vi "Get Summary.vi"(7 "Style":enum16{"Diff", "Plain"}(ring), 8 "error in (no error)":errorcluster, 10 "Item":string, 11 "Result Model by Reference In":refnum<class "Result Model.lvclass">) -> (0 "error out":errorcluster, 2 "Summary":string)   [LabVIEW 2020, in "Result Model.lvclass"]
uses:
  Result Model.lvclass
  Result Model.lvclass/Result Model.ctl
  Framework/Utilities/Utilities.lvlib
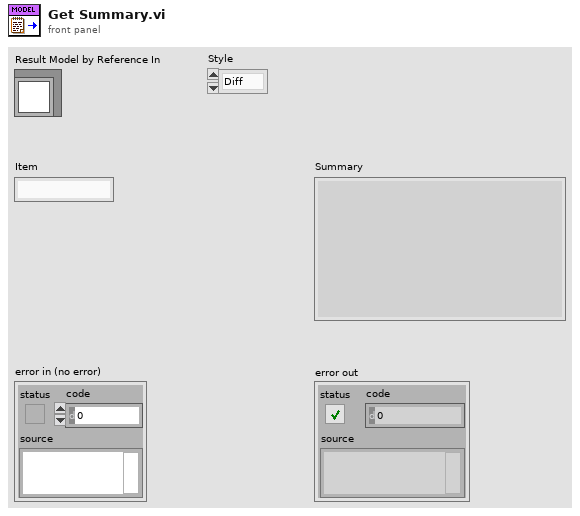
[diagram p1: front panel]
types:
  T1 = typedef "Result Model.lvclass/Statistics.ctl" = cluster{"Method Count":u32, "Executed Methods":u32, "Passed Methods":u32, "Failed Methods":u32, "Method Errors":u32, "Skipped Method":u32, "Progress [%]":dbl}
  T2 = typedef "Result.lvlib/Status.ctl" = enum16{"", "Passed", "Failed", "Error", "Skipped", "Setup Error", "Broken", "Teardown Error"}
  T3 = typedef "Result.lvlib/Type.ctl" = enum16{"Test Case", "Test Suite", "Test Run", "Pass", "Fail", "Skip", "Pass if", "Fail if", "Pass if Error", "Fail if Error", "Pass if Equal", "Fail if Equal"}
  T4 = cluster{"Tests":string[], "Run Queue":string[], "Test Statuses":map{string, T2}, "Execution Time":map{string, dbl}, "Assertions":map{string, cluster{"Result Type":T3, "Status":T2, "Description":string, "Data":cluster{"Expected":variant, "Actual":variant, "Delta":variant}}[]}}
  T5 = map{string, cluster{"Result Type":T3, "Status":T2, "Description":string, "Data":cluster{"Expected":variant, "Actual":variant, "Delta":variant}}[]}
  T6 = cluster{"Result Type":T3, "Status":T2, "Description":string, "Data":cluster{"Expected":variant, "Actual":variant, "Delta":variant}}[]
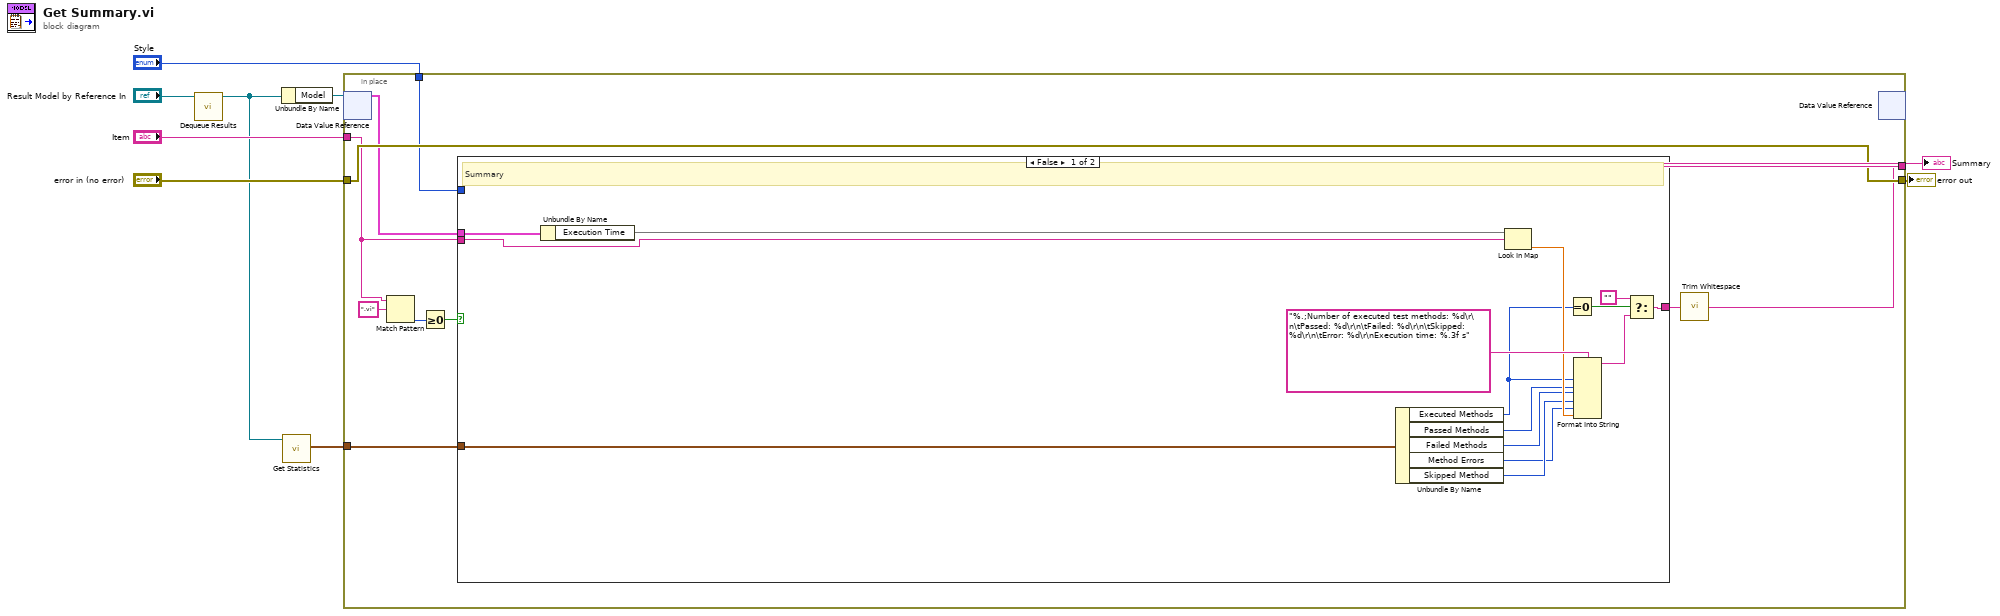
[diagram p0: block diagram]
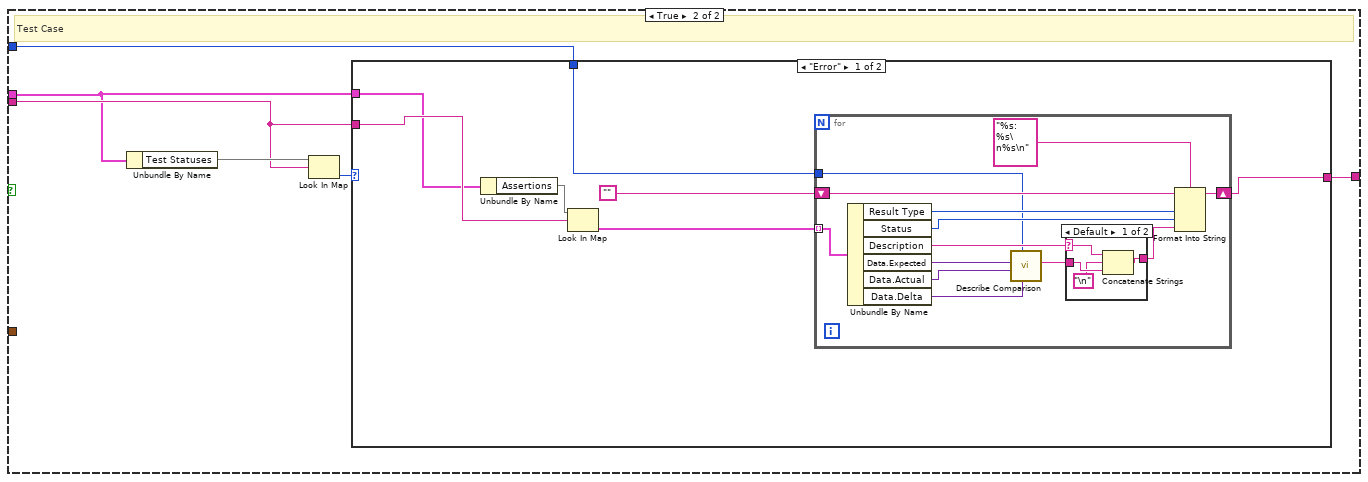
[diagram p2: hidden frame]
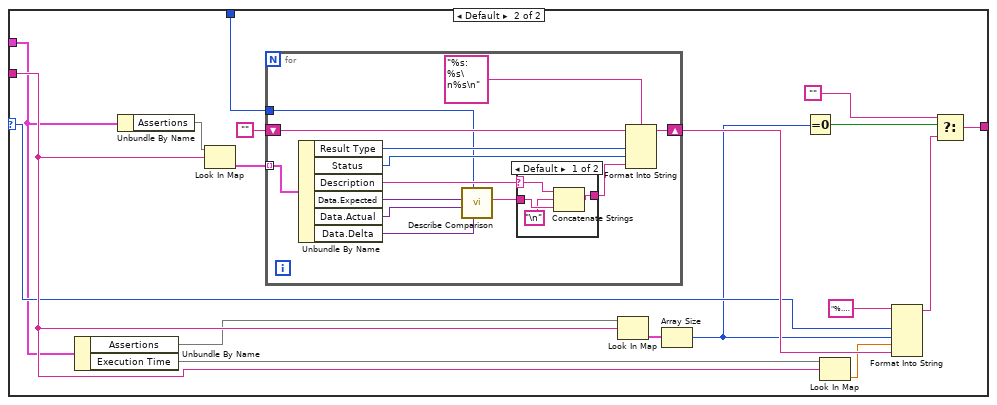
[diagram p4: hidden frame]
diagram:
  n1 = call "Dequeue Results.vi"("Result Model by Reference in"="Result Model by Reference In") -> ("Result Model by Reference out"=w1:refnum<class "Result Model.lvclass">)  [unwired: 10 in]
  n2 = Unbundle By Name(w1) -> ("Model"=w9:refnum<data-value>)
  n3 = call "Get Statistics.vi"("Result Model in"=w1) -> ("Results"=w2:T1)  [unwired: 9 in, 1 out]
  n4 = in-place {
    in-place-border: "error in (no error)" -> [w19]
    in-place-border: [w19] -> w5
    in-place-border: "Item" -> [w17]
    in-place-border: [w16] -> w4
    in-place-border: "Style" -> [w15]
    in-place-border: w2 -> [w10]
    n5 = in-place-dvr #1(w9) -> (w18:T4)  [unwired: 1 out]
    n6 = Match Pattern(string=w17, regular expression=".vi") -> (offset past match=w12:i32)  [unwired: 1 in, 3 out]
    n7 = Greater Or Equal To 0?(x=w12) -> (x >= 0?=w13:bool)
    n8 = case shown="False" w13 {
      tunnel: w17 -> [w20 w37]
      tunnel: [w29 w39] -> w14
      tunnel: w18 -> [w26 w36]
      tunnel: w15 -> [_ w35]
      tunnel: w10 -> [w21 _]
      frame False {
        # "Summary"
        n9 = Unbundle By Name(w26) -> ("Execution Time"=w27:map{string, dbl})
        n10 = Unbundle By Name(w21) -> ("Executed Methods"=w32:u32, "Passed Methods"=w25:u32, "Failed Methods"=w24:u32, "Method Errors"=w22:u32, "Skipped Method"=w23:u32)
        n11 = Look In Map(map=w27, key=w20) -> (value=w33:dbl)  [unwired: 1 in, 1 out]
        n12 = Equal To 0?(x=w32) -> (x = 0?=w31:bool)
        n13 = Format Into String(format string="%.;Number of executed test methods: %d\r\n\tPassed: %d\r\n\tFailed: %d\r\n\tSkipped: %d\r\n\tError: %d\r\nExecution time: %.3f s", w32, w25, w24, w23, w22, w33) -> (resulting string=w30:string)  [unwired: 2 in, 1 out]
        n14 = Select(t="", s=w31, f=w30) -> (s? t:f=w29:string)
      }
      frame True {
        # "Test Case"
        n15 = Unbundle By Name(w36) -> ("Test Statuses"=w38:map{string, T2})
        n16 = Look In Map(map=w38, key=w37) -> (value=w40:T2)  [unwired: 1 in, 1 out]
        n17 = case shown="\"Error\"" w40 {
          selector: w40 -> [_ w74]
          tunnel: [w46 w81] -> w39
          tunnel: w37 -> [w47 w79]
          tunnel: w36 -> [w44 w69]
          tunnel: w35 -> [w45 w70]
          frame "Error" {
            n18 = Unbundle By Name(w44) -> ("Assertions"=w42:T5)
            n19 = Look In Map(map=w42, key=w47) -> (value=w41:T6)  [unwired: 1 in, 1 out]
            n20 = for {
              tunnel: w41 -> [w59] mode=indexing
              shift-right: [w54] -> w46
              shift-left: "" -> [w55]
              tunnel: w45 -> [w48]
              n21 = Unbundle By Name(w59) -> ("Result Type"=w52:T3, "Status"=w51:T2, "Description"=w49:string, "Data.Expected"=w58:variant, "Data.Actual"=w57:variant, "Data.Delta"=w56:variant)
              n22 = call "Describe Comparison.vi"("Delta"=w56, "Style"=w48, "Actual"=w57, "Expected"=w58) -> ("Description"=w53:string)  [unwired: 7 in]
              n23 = case shown="Default" w49 {
                selector: w49 -> [w63 _]
                tunnel: w53 -> [w62 w65]
                tunnel: [w64 w65] -> w50
                frame Default {
                  n24 = Concatenate Strings(w63, "\n", w62) -> (w64:string)
                }
                frame "" {
                }
              }
              n25 = Format Into String(format string="%s: %s\n%s\n", initial string=w55, w52, w51, w50) -> (resulting string=w54:string)  [unwired: 1 in, 1 out]
            }
          }
          frame Default {
            n26 = Unbundle By Name(w69) -> ("Assertions"=w77:T5, "Execution Time"=w78:map{string, dbl})
            n27 = Unbundle By Name(w69) -> ("Assertions"=w67:T5)
            n28 = Look In Map(map=w67, key=w79) -> (value=w66:T6)  [unwired: 1 in, 1 out]
            n29 = for {
              tunnel: w66 -> [w95] mode=indexing
              shift-right: [w90] -> w75
              shift-left: "" -> [w91]
              tunnel: w70 -> [w84]
              n30 = Unbundle By Name(w95) -> ("Result Type"=w88:T3, "Status"=w87:T2, "Description"=w85:string, "Data.Expected"=w94:variant, "Data.Actual"=w93:variant, "Data.Delta"=w92:variant)
              n31 = call "Describe Comparison.vi"("Delta"=w92, "Style"=w84, "Actual"=w93, "Expected"=w94) -> ("Description"=w89:string)  [unwired: 7 in]
              n32 = case shown="Default" w85 {
                selector: w85 -> [w99 _]
                tunnel: w89 -> [w98 w101]
                tunnel: [w100 w101] -> w86
                frame Default {
                  n33 = Concatenate Strings(w99, "\n", w98) -> (w100:string)
                }
                frame "" {
                }
              }
              n34 = Format Into String(format string="%s: %s\n%s\n", initial string=w91, w88, w87, w86) -> (resulting string=w90:string)  [unwired: 1 in, 1 out]
            }
            n35 = Look In Map(map=w77, key=w79) -> (value=w83:T6)  [unwired: 1 in, 1 out]
            n36 = Array Size(array=w83) -> (size(s)=w73:i32)
            n37 = Equal To 0?(x=w73) -> (x = 0?=w82:bool)
            n38 = Look In Map(map=w78, key=w79) -> (value=w72:dbl)  [unwired: 1 in, 1 out]
            n39 = Format Into String(format string="%.;%s, Assertions: %d, Execution time: %.3f \n\n%s", w74, w73, w72, w75) -> (resulting string=w76:string)  [unwired: 2 in, 1 out]
            n40 = Select(t="", s=w82, f=w76) -> (s? t:f=w81:string)
          }
        }
      }
    }
    n41 = call <vilib>:"Trim Whitespace.vi"("string"=w14) -> ("trimmed string"=w16:string)  [unwired: 1 in]
    n42 = in-place-dvr #1() -> ()  [unwired: 1 in, 2 out]
  }
  "Summary" <- w4
  "error out" <- w5
